vi "UTF-8 Path Probe.vi"(11 "UTF-8 Path":refnum<class "UTF-8 Path.lvclass">) -> (2 "Value String":string, 3 "Boolean":bool)   [LabVIEW 2020, in "G-Unicode.lvlib" / "UTF-8 Path.lvclass"]
uses:
  UTF-8 Path.lvclass
  G-Unicode.lvlib
  Unicode/Controls/String Encoding.ctl
panel:
  out "Unicode":string
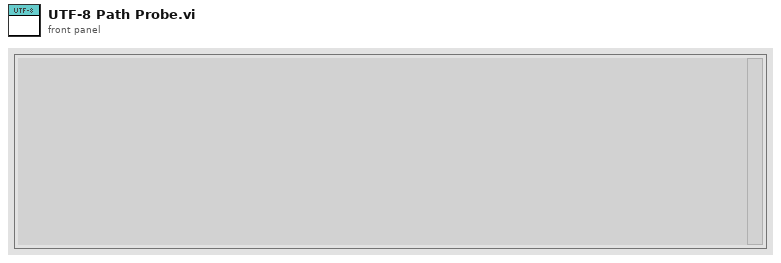
[diagram p1: front panel]
types:
  T1 = typedef "G-Unicode.lvlib/String Encoding.ctl" = enum16{"ANSI", "UTF-8", "UTF-16LE", "UTF-16BE", "Unknown"}
  T2 = typedef "G-Unicode.lvlib/Encoded UTF-8 Path.ctl" = path
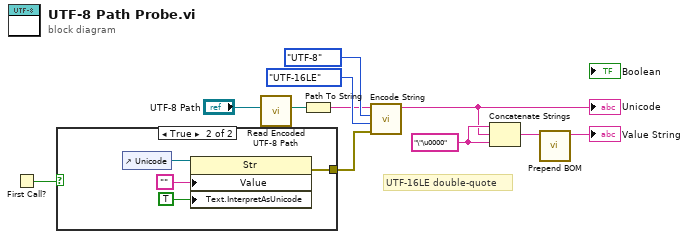
[diagram p0: block diagram]
diagram:
  w4 = "\"\u0000" ("string")
  # "UTF-16LE double-quote"
  n1 = First Call?() -> (First Call?: T/F=w1:bool)
  n2 = case shown="True" w1 {
    tunnel: [_ w15] -> w11
    frame False {
    }
    frame True {
      n3 = control-ref of="Unicode"() -> (w12:refnum<vi>)
      n4 = property on="Property Node" class="Str"(reference=w12, "Value"="", "Text.InterpretAsUnicode"=TRUE ("Force Unicode Text")) -> (error out=w15:errorcluster)  [unwired: 1 in, 1 out]
    }
  }
  n5 = call "Read Encoded UTF-8 Path.vi"("UTF-8 Path"="UTF-8 Path") -> ("Encoded UTF-8 Path"=w8:T2)  [unwired: 10 in]
  n6 = Path To String(path=w8) -> (string=w6:string)
  n7 = call "Encode String.vi"("error in"=w11, "Output Encoding (UTF-16LE)"=String_Encoding."UTF-16LE" ("Output Encoding (UTF-8)"), "Input Encoding (ANSI)"=String_Encoding."UTF-8", "String in"=w6) -> ("String out"=w3:string)  [unwired: 6 in, 1 out]
  "Unicode" <- w3
  n8 = Concatenate Strings(w4, w3, w4) -> (w2:string)
  n9 = call "Prepend BOM.vi"("String"=w2) -> ("String with BOM"=→"Value String":string)  [unwired: 9 in, 1 out]
